vi "Bidirectional Streaming RouteGuide Test.vi"() -> ()   [LabVIEW 2019, in "route_guide_client.lvlib"]
uses:
  route_guide_client.lvlib
  RPC Messages/routeguide_RouteNote.ctl
  RPC Messages/routeguide_Point.ctl
  <vilib>/gRPC/LabVIEW gRPC Library/grpc-lvsupport-release.lvlib
panel:
  in  "error in":errorcluster
  out "error out":errorcluster
  out "Response Data":T1[](array[typedef])
  in  "Request Data":T1[](array[typedef])=[{"location"={"latitude"=1, "longitude"=1}, "message"="Point 1"}, {"location"={"latitude"=2, "longitude"=2}, "message"="Point 2"}]
  in  "Server Address":string="localhost:50051"
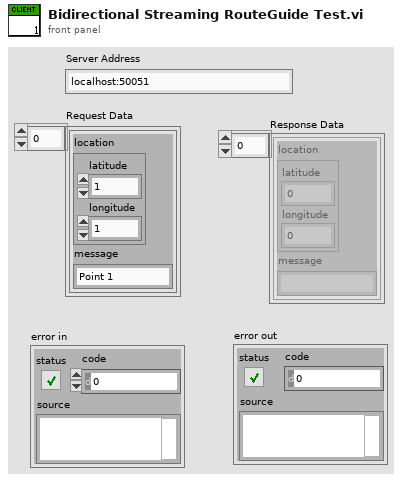
[diagram p1: front panel]
types:
  T1 = typedef "route_guide_client.lvlib/routeguide_RouteNote.ctl" = cluster{"location":T2, "message":string}
  T2 = typedef "route_guide_client.lvlib/routeguide_Point.ctl" = cluster{"latitude":i32, "longitude":i32}
  T3 = typedef "grpc-lvsupport-release.lvlib/grpcId.ctl" = u64
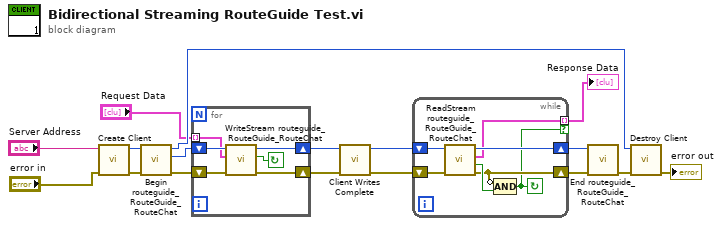
[diagram p0: block diagram]
diagram:
  n1 = call "Create Client.vi"("error in"="error in", "address"="Server Address") -> ("error out"=w15:errorcluster, "gRPC ID Out"=w16:T3)  [unwired: 8 in]
  n2 = call "Begin routeguide_RouteGuide_RouteChat.vi"("error in"=w15, "gRPC ID"=w16) -> ("error out"=w13:errorcluster, "Call Id Out"=w14:T3, "gRPC ID out"=w11:T3)  [unwired: 7 in]
  n3 = for {
    shift-right: [w20] -> w6
    shift-left: w14 -> [w23]
    shift-right: [w19] -> w4
    shift-left: w13 -> [w22]
    tunnel: "Request Data" -> [w21] mode=indexing
    stop <- w18 continue-if-true
    n4 = call "WriteStream routeguide_RouteGuide_RouteChat.vi"("error in"=w22, "Request Data"=w21, "Call ID in"=w23) -> ("error out"=w19:errorcluster, "Success"=w18:bool, "Call ID"=w20:T3)  [unwired: 6 in]
  }
  n5 = call <vilib>:"Client Writes Complete.vi"("error in"=w4, "ClientID in"=w6) -> ("error out"=w3:errorcluster, "ClientID out"=w5:T3)  [unwired: 8 in]
  n6 = while {
    shift-right: [w26] -> w9
    shift-left: w5 -> [w29]
    shift-right: [w27] -> w8
    shift-left: w3 -> [w28]
    tunnel: [w25] -> w7 mode=indexing if=w24
    stop <- w24 continue-if-true
    n7 = call "ReadStream routeguide_RouteGuide_RouteChat.vi"("error in"=w28, "Call ID in"=w29) -> ("error out"=w27:errorcluster, "Success"=w30:bool, "Response Data"=w25:T1, "Call ID"=w26:T3)  [unwired: 6 in]
    n8 = Compound Arithmetic op=AND(invert w27, w30) -> (w24:bool)
  }
  "Response Data" <- w7
  n9 = call "End routeguide_RouteGuide_RouteChat.vi"("error in"=w8, "Call ID in"=w9) -> ("error out"=w12:errorcluster)  [unwired: 8 in, 1 out]
  n10 = call "Destroy Client.vi"("error in"=w12, "gRPC ID"=w11) -> ("error out"=→"error out":errorcluster)  [unwired: 9 in]
